vi "Detailsd Update Report.vi"() -> (3 "appended array":string[](array[string]))   [LabVIEW 2021]
uses:
  controls/Read_Update.ctl
  Template/Main_VI/Control/Ini.ctl
panel:
  out "error in (no error) 3":errorcluster
  out "Part No":string
  out "Serial  No":string
  out "Rev":string
  out "Test Type":string
  out "Operator":string
  out "Result":string
  out "Time stamp":string
  out "Start Time":string
  out "date/time string 2":string
  out "date/time string":string
  out "Serial Number":string
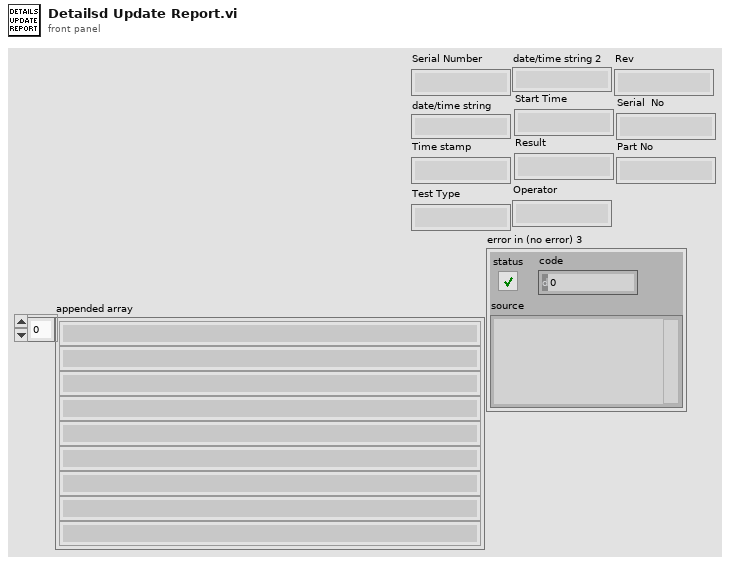
[diagram p1: front panel]
types:
  T1 = typedef "Read_Update.ctl" = enum16{"Read", "Update", "Exit"}
  T2 = typedef "Ini.ctl" = enum16{"Write", "Read"}
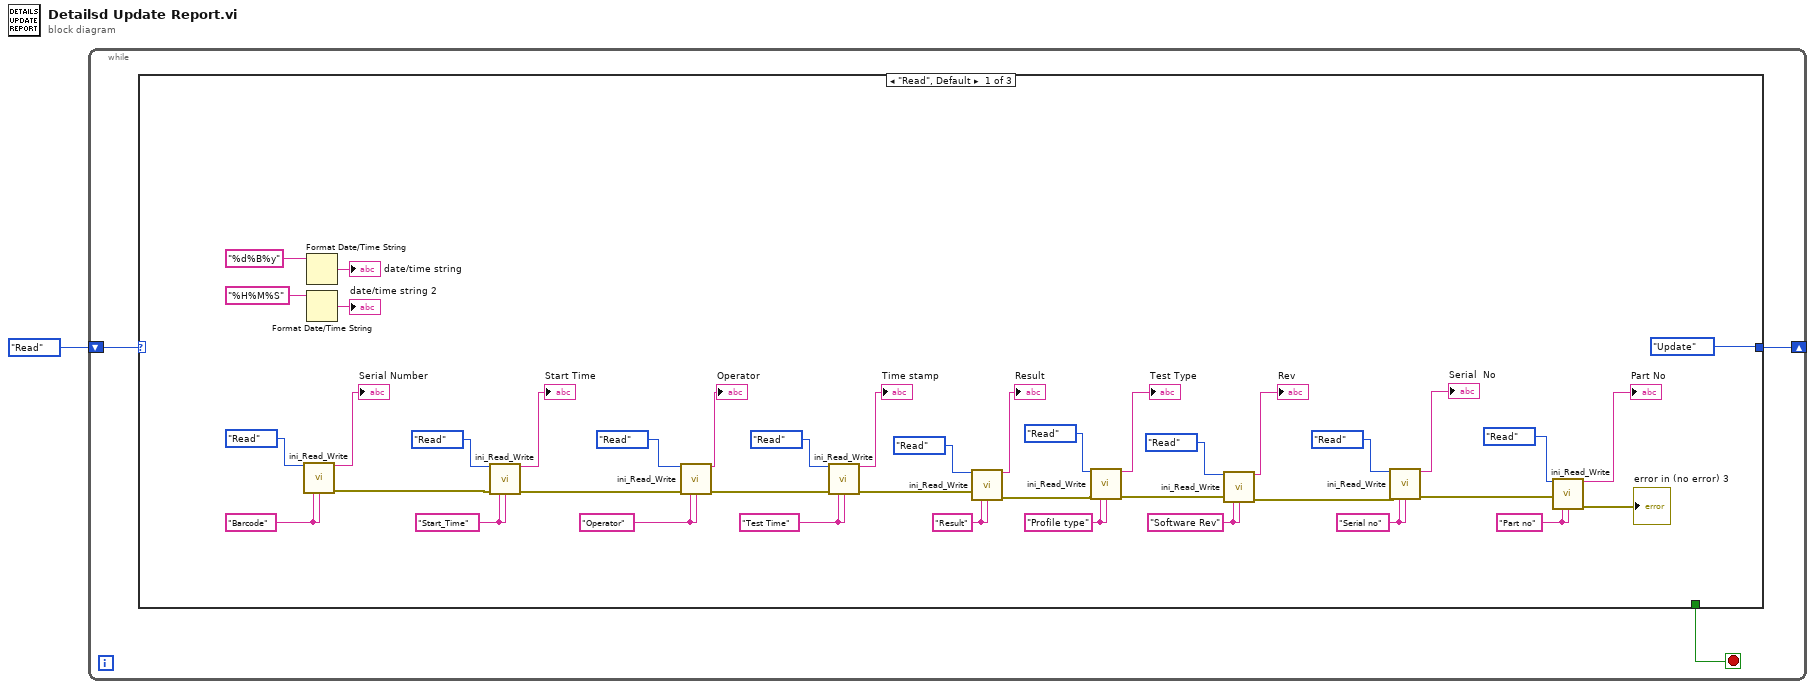
[diagram p0: block diagram]
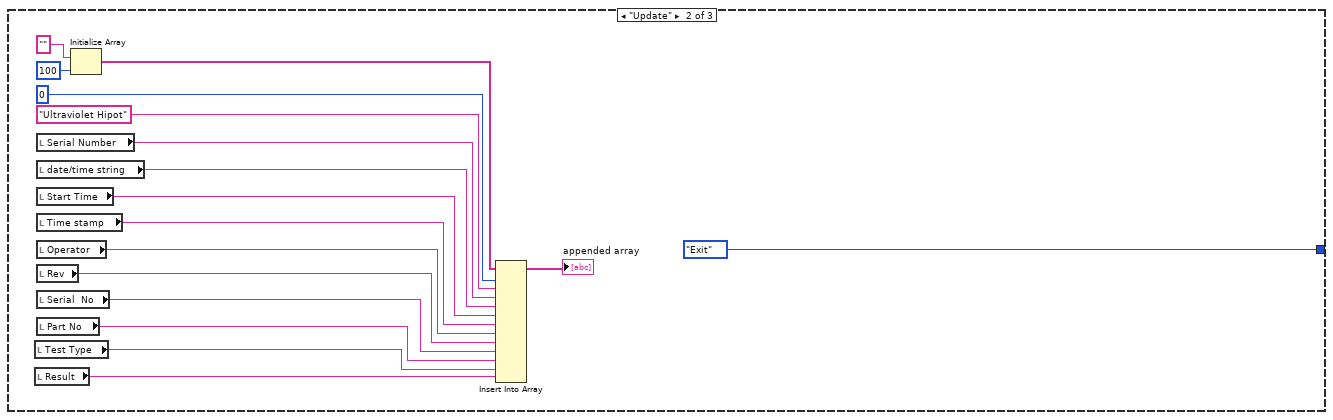
[diagram p2: hidden frame]
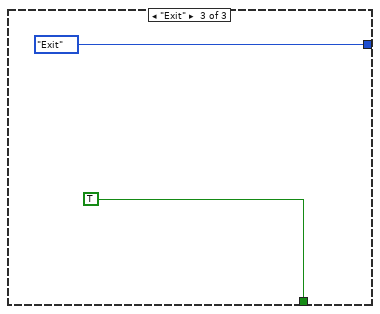
[diagram p3: hidden frame]
diagram:
  n1 = while {
    shift-right: [w3] -> _
    shift-left: Read_Update."Read" -> [w4]
    stop <- w2 stop-if-true
    n2 = case shown="\"Read\", Default" w4 {
      tunnel: [Read_Update."Update" Read_Update."Exit" Read_Update."Exit"] -> w3
      tunnel: [_ _ TRUE] -> w2
      frame "Read", Default {
        w13 = "Part no" ("Read Section")
        w18 = "Serial no" ("Write Section")
        w20 = "Software Rev" ("Write Section")
        w5 = "Profile type" ("Write key")
        w22 = "Test Time" ("Write Section")
        w23 = "Operator" ("Write Section")
        w29 = "Result" ("Read Section")
        w30 = "Start_Time" ("Read Section")
        w31 = "Barcode" ("Read Section")
        n3 = call "ini_Read_Write.vi"(0:Ini."Read", "Read Section"=w31, "Read Key"=w31) -> ("value"=→"Serial Number":string, "error in (no error) 3"=w35:errorcluster)  [unwired: 11 in]
        n4 = Format Date/Time String(time format string (%c)="%d%B%y") -> (date/time string=→"date/time string":string)  [unwired: 2 in]
        n5 = Format Date/Time String(time format string (%c)="%H%M%S") -> (date/time string=→"date/time string 2":string)  [unwired: 2 in]
        n6 = call "ini_Read_Write.vi"(0:Ini."Read", "error in (no error) 2"=w35, "Read Section"=w30, "Read Key"=w30) -> ("value"=→"Start Time":string, "error in (no error) 3"=w27:errorcluster)  [unwired: 10 in]
        n7 = call "ini_Read_Write.vi"(0:Ini."Read", "error in (no error) 2"=w27, "Read Section"=w23, "Read Key"=w23) -> ("value"=→"Operator":string, "error in (no error) 3"=w26:errorcluster)  [unwired: 10 in]
        n8 = call "ini_Read_Write.vi"(0:Ini."Read", "error in (no error) 2"=w26, "Read Section"=w22, "Read Key"=w22) -> ("value"=→"Time stamp":string, "error in (no error) 3"=w24:errorcluster)  [unwired: 10 in]
        n9 = call "ini_Read_Write.vi"(0:Ini."Read", "error in (no error) 2"=w24, "Read Section"=w29, "Read Key"=w29) -> ("value"=→"Result":string, "error in (no error) 3"=w7:errorcluster)  [unwired: 10 in]
        n10 = call "ini_Read_Write.vi"(0:Ini."Read", "error in (no error) 2"=w7, "Read Section"=w5, "Read Key"=w5) -> ("value"=→"Test Type":string, "error in (no error) 3"=w6:errorcluster)  [unwired: 10 in]
        n11 = call "ini_Read_Write.vi"(0:Ini."Read", "error in (no error) 2"=w6, "Read Section"=w20, "Read Key"=w20) -> ("value"=→"Rev":string, "error in (no error) 3"=w15:errorcluster)  [unwired: 10 in]
        n12 = call "ini_Read_Write.vi"(0:Ini."Read", "error in (no error) 2"=w15, "Read Section"=w18, "Read Key"=w18) -> ("value"=→"Serial  No":string, "error in (no error) 3"=w16:errorcluster)  [unwired: 10 in]
        n13 = call "ini_Read_Write.vi"(0:Ini."Read", "error in (no error) 2"=w16, "Read Section"=w13, "Read Key"=w13) -> ("value"=→"Part No":string, "error in (no error) 3"=→"error in (no error) 3":errorcluster)  [unwired: 10 in]
      }
      frame "Update" {
        n14 = local read "Test Type"() -> (w46:string)
        n15 = local read "Result"() -> (w49:string)
        n16 = local read "Serial Number"() -> (w60:string)
        n17 = local read "date/time string"() -> (w59:string)
        n18 = local read "Start Time"() -> (w57:string)
        n19 = local read "Time stamp"() -> (w56:string)
        n20 = local read "Operator"() -> (w55:string)
        n21 = local read "Rev"() -> (w50:string)
        n22 = local read "Serial  No"() -> (w48:string)
        n23 = local read "Part No"() -> (w47:string)
        n24 = Initialize Array("" ("string"), 100 ("dimension size")) -> (w51:string[])
        n25 = Insert Into Array(array=w51, index=0, new element #1="Ultraviolet Hipot" ("string"), new element #2=w60, new element #3=w59, new element #4=w57, new element #5=w56, new element #6=w55, new element #7=w50, new element #8=w48, new element #9=w47, new element #10=w46, new element #11=w49) -> (→"appended array":string[])
      }
      frame "Exit" {
      }
    }
  }
